vi "Read SM.vi"(8 "error in (no error)":errorcluster, 10 "Vo":dbl, 11 "Puerto serial":refnum<visa-resource-name>) -> (0 "error out":errorcluster, 3 "Acquistion Data":T1)   [LabVIEW 2020]
uses:
  39de7056-9ed4-47ec-a934-0fe14cb6d8de.vi
  68284e2b-69f7-4644-8932-20630b6eccd7.vi
  controls/Acquisition data --typedef.ctl
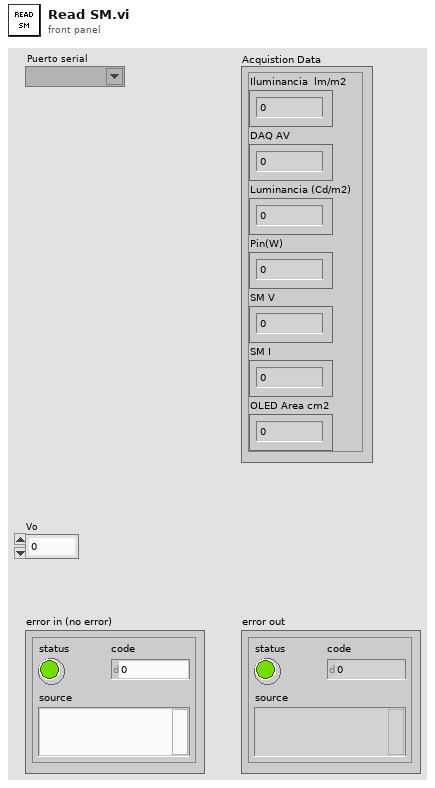
[diagram p1: front panel]
types:
  T1 = typedef "Acquisition data --typedef.ctl" = cluster{"Iluminancia  lm/m2":dbl, "DAQ AV":dbl, "Luminancia (Cd/m2)":dbl, "Pin(W)":dbl, "SM V":dbl, "SM I":dbl, "OLED Area cm2":dbl}
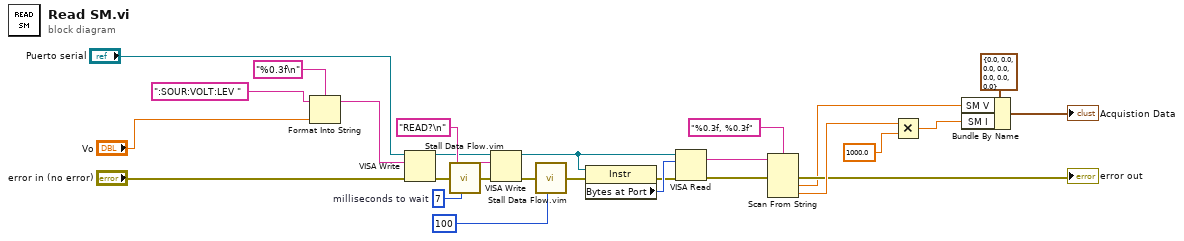
[diagram p0: block diagram]
diagram:
  w23 = u32 7  # milliseconds to wait
  n1 = Format Into String(format string="%0.3f\n", initial string=":SOUR:VOLT:LEV " ("Comando"), "Vo") -> (resulting string=w2:string)  [unwired: 1 in, 1 out]
  n2 = VISA Write(VISA resource name="Puerto serial", write buffer=w2, error in (no error)="error in (no error)") -> (VISA resource name out=w19:refnum<visa-resource-name>, error out=w18:errorcluster)  [unwired: 1 out]
  n3 = call "Stall Data Flow.vim"("value in"=w18, "milliseconds to wait"=w23) -> ("value out"=w20:errorcluster)  [unwired: 1 out]
  n4 = VISA Write(VISA resource name=w19, write buffer="READ?\n" ("Comando"), error in (no error)=w20) -> (VISA resource name out=w26:refnum<visa-resource-name>, error out=w21:errorcluster)  [unwired: 1 out]
  n5 = call "Stall Data Flow.vim"("value in"=w21, "milliseconds to wait"=u32 100) -> ("value out"=w22:errorcluster)  [unwired: 1 out]
  n6 = property class="Instr"(reference=w26, error in=w22) -> (error out=w25:errorcluster, "Bytes at Port"=w27:u32)  [unwired: 1 out]
  n7 = VISA Read(VISA resource name=w26, byte count=w27, error in (no error)=w25) -> (read buffer=w14:string, error out=w15:errorcluster)  [unwired: 2 out]
  n8 = Scan From String(format string="%0.3f, %0.3f", input string=w14, error in=w15) -> (error out=→"error out":errorcluster, output 1=w8:dbl, output 2=w12:dbl)  [unwired: 3 in, 2 out]
  n9 = Multiply(x=w12, y=1000.0) -> (x*y=w7:dbl)
  n10 = Bundle By Name(cluster=T1 {"Iluminancia  lm/m2"=0.0, "DAQ AV"=0.0, "Luminancia (Cd/m2)"=0.0, "Pin(W)"=0.0, "SM V"=0.0, "SM I"=0.0, "OLED Area cm2"=0.0} ("Acquistion Data"), "SM V"=w8, "SM I"=w7) -> (→"Acquistion Data":T1)
